vi "Shuffle Array 1D Template.vi"(0 "Array In":variant[](array[variant])) -> (2 "Shuffled Array":variant[](array[variant]))   [LabVIEW 2012]
doc: "Shuffles the elements of the input array into a random order. For 2D arrays can shuffle rows, columns or individual elements depending on the rank input."
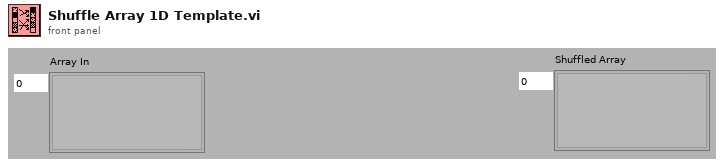
[diagram p1: front panel]
types:
  T1 = cluster{"number: 0 to 1":dbl, "Variant":variant}[]
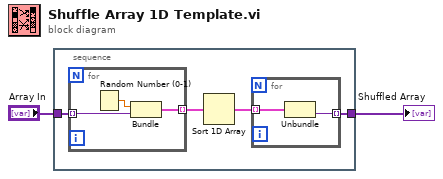
[diagram p0: block diagram]
diagram:
  n1 = stacked-sequence {
    tunnel: "Array In" -> [w6]
    tunnel: [w5] -> w1
    frame #0 {
      n2 = for {
        tunnel: w6 -> [w10] mode=indexing
        tunnel: [w9] -> w4 mode=indexing
        n3 = Random Number (0-1)() -> (number: 0 to 1=w11:dbl)
        n4 = Bundle("number: 0 to 1"=w11, "Variant"=w10) -> (w9:cluster{"number: 0 to 1":dbl, "Variant":variant})  [unwired: 1 out]
      }
      n5 = Sort 1D Array(array=w4) -> (sorted array=w3:T1)
      n6 = for {
        tunnel: w3 -> [w8] mode=indexing
        tunnel: [w7] -> w5 mode=indexing
        n7 = Unbundle(w8) -> ("Variant"=w7:variant)  [unwired: 1 out]
      }
    }
  }
  "Shuffled Array" <- w1
